vi "testUIPanelOpenifpreviouslyOpen.vi"(8 "error in (no error)":errorcluster, 11 "testStateMachineUtilities in":refnum<class "testStateMachineUtilities.lvclass">) -> (0 "error out":errorcluster, 3 "testStateMachineUtilities out":refnum<class "testStateMachineUtilities.lvclass">)   [LabVIEW 2020, in "testStateMachineUtilities.lvclass"]
uses:
  testStateMachineUtilities.lvclass
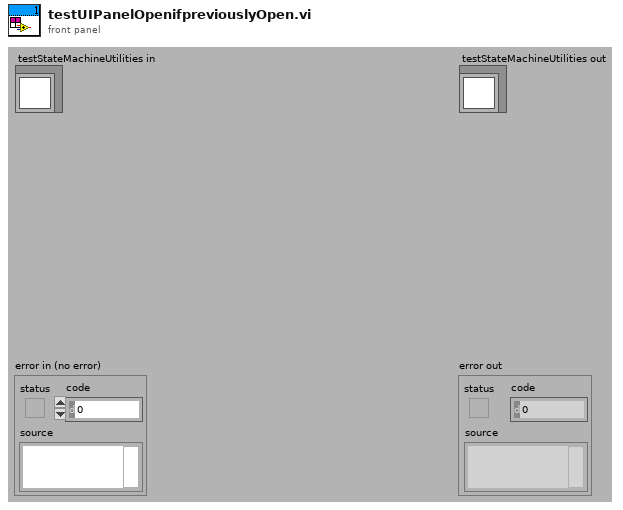
[diagram p1: front panel]
types:
  T1 = enum32{"Bad", "Idle", "Run top level", "Running"}
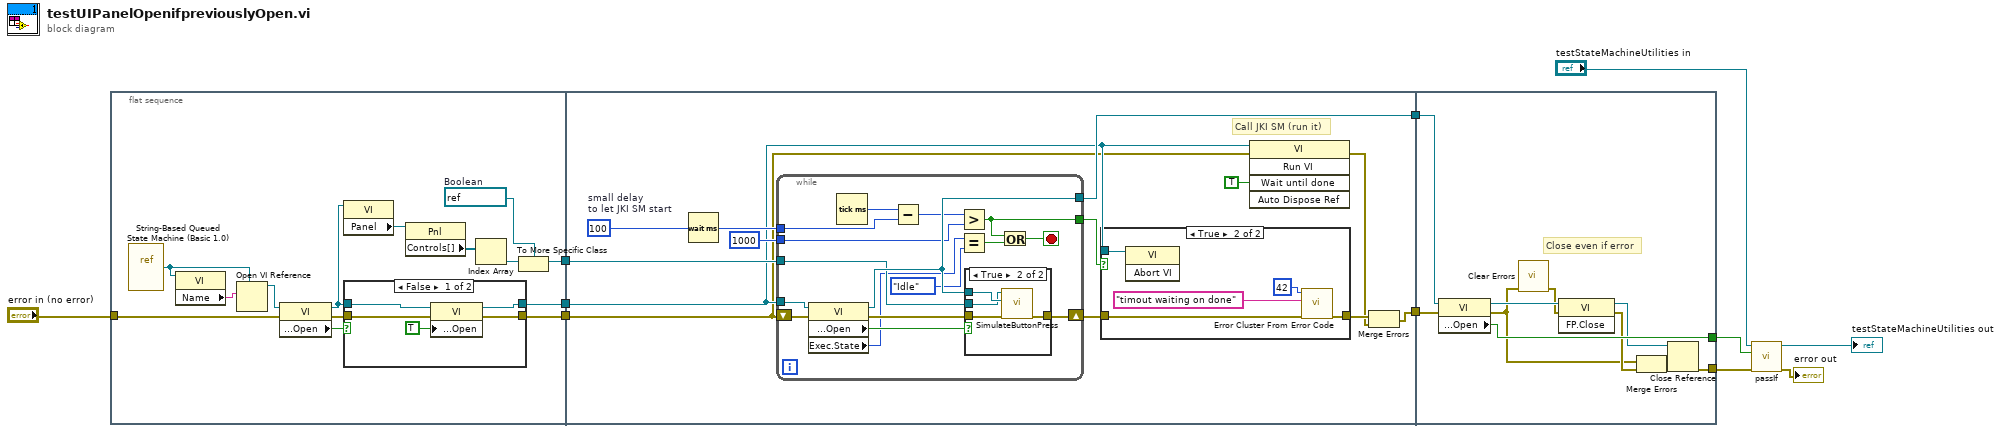
[diagram p0: block diagram]
diagram:
  n1 = flat-sequence {
    tunnel: [w23] -> w8
    tunnel: [w22] -> w3
    tunnel: "error in (no error)" -> [w21]
    tunnel: [w15] -> w1
    tunnel: w8 -> [w37]
    tunnel: [w45] -> w7
    tunnel: [w34] -> w4
    tunnel: w3 -> [w35]
    tunnel: w1 -> [w44]
    tunnel: w7 -> [w82]
    tunnel: [w80] -> w6
    tunnel: [w76] -> w5
    tunnel: w4 -> [w81]
    frame #0 {
      w16 = refnum<vi> refnum  # Boolean
      n2 = vi-ref "String-Based Queued State Machine (Basic 1.0).vi"() -> (w13:refnum<vi>)
      n3 = property class="VI"(reference=w13) -> ("Name"=w14:string)  [unwired: 1 in, 2 out]
      n4 = Open VI Reference(type specifier VI Refnum (for type only)=w13, vi path=w14) -> (vi reference=w12:refnum<vi>)  [unwired: 4 in, 1 out]
      n5 = property class="VI"(reference=w12, error in=w21) -> (reference out=w20:refnum<vi>, error out=w25:errorcluster, "Front Panel.Open"=w24:bool)
      n6 = property class="VI"(reference=w20) -> ("Panel"=w19:refnum<vi>)  [unwired: 1 in, 2 out]
      n7 = case shown="False" w24 {
        tunnel: w20 -> [w30 w32]
        tunnel: w25 -> [w28 w31]
        tunnel: [w27 w32] -> w23
        tunnel: [w26 w31] -> w22
        frame False {
          n8 = property class="VI"(reference=w30, error in=w28, "Front Panel.Open"=TRUE ("Front Panel Window:Open")) -> (reference out=w27:refnum<vi>, error out=w26:errorcluster)
        }
        frame True {
        }
      }
      n9 = property class="Pnl"(reference=w19) -> ("Controls[]"=w18:refnum<vi>[])  [unwired: 1 in, 2 out]
      n10 = Index Array(array=w18) -> (element=w17:refnum<vi>)  [unwired: 1 in]
      n11 = To More Specific Class(target class=w16, reference=w17) -> (specific class reference=w15:refnum<vi>)  [unwired: 1 in, 1 out]
    }
    frame #1 {
      w43 = u32 100  # small delay to let JKI SM start
      # "Call JKI SM (run it)"
      n12 = Wait (ms)(milliseconds to wait=w43) -> (millisecond timer value=w42:u32)
      n13 = while {
        tunnel: w37 -> [w67]
        tunnel: [w63] -> w45
        shift-right: [w66] -> w39
        shift-left: w35 -> [w65]
        tunnel: w44 -> [w62]
        tunnel: w42 -> [w60]
        tunnel: u32 1000 ("milliseconds to wait") -> [w58]
        tunnel: [w55] -> w40
        stop <- w56 stop-if-true
        n14 = property class="VI"(reference=w67, error in=w65) -> (reference out=w63:refnum<vi>, error out=w64:errorcluster, "Front Panel.Open"=w57:bool, "Exec.State"=w54:T1)
        n15 = Tick Count (ms)() -> (millisecond timer value=w61:u32)
        n16 = Subtract(x=w61, y=w60) -> (x-y=w59:u32)
        n17 = Greater?(x=w59, y=w58) -> (0:w55:bool)
        n18 = Equal?(x=w54, y=T1."Idle" ("Execution:State")) -> (x = y?=w52:bool)
        n19 = case shown="True" w57 {
          tunnel: [w68 w70] -> w66
          tunnel: w64 -> [w68 w69]
          tunnel: w63 -> [_ w72]
          tunnel: w62 -> [_ w71]
          frame False {
          }
          frame True {
            n20 = call "SimulateButtonPress.vi"("error in (no error)"=w69, "VIRef"=w72, "BooleanCtrlRef"=w71) -> ("error out"=w70:errorcluster)  [unwired: 8 in]
          }
        }
        n21 = Or(x=w55, y=w52) -> (x .or. y?=w56:bool)
      }
      n22 = case shown="True" w40 {
        tunnel: w37 -> [_ w51]
        tunnel: w39 -> [w46 w50]
        tunnel: [w46 w49] -> w38
        frame False {
        }
        frame True {
          n23 = invoke class="VI" method="Abort VI"(reference=w51) -> ()  [unwired: 2 in, 3 out]
          n24 = call <vilib>:"Error Cluster From Error Code.vi"("error in (no error)"=w50, "error message (\"\")"="timout waiting on done" ("error message (\"\")"), "error code (0)"=42) -> ("error out"=w49:errorcluster)  [unwired: 6 in]
        }
      }
      n25 = invoke class="VI" method="Run VI"(reference=w37, error in=w35, "Wait until done"=TRUE ("Wait Until Done")) -> (error out=w33:errorcluster)  [unwired: 2 in, 4 out]
      n26 = Merge Errors(w38, w33) -> (w34:errorcluster)
    }
    frame #2 {
      # "Close even if error"
      n27 = property class="VI"(reference=w82, error in=w81) -> (reference out=w79:refnum<vi>, error out=w74:errorcluster, "Front Panel.Open"=w80:bool)
      n28 = call <vilib>:"Clear Errors.vi"("error in (no error)"=w74) -> ("error out"=w73:errorcluster)  [unwired: 5 in, 1 out]
      n29 = invoke class="VI" method="FP.Close"(reference=w79, error in=w73) -> (reference out=w78:refnum<vi>, error out=w77:errorcluster)  [unwired: 1 in, 1 out]
      n30 = Merge Errors(w74, w77) -> (w75:errorcluster)
      n31 = Close Reference(reference=w78, error in (no error)=w75) -> (error out=w76:errorcluster)
    }
  }
  n32 = call-dynamic "passIf.vi"("error in (no error)"=w5, "pass"=w6, "TestCase in"="testStateMachineUtilities in") -> ("error out"=→"error out":errorcluster, "TestCase out"=→"testStateMachineUtilities out":refnum<class "testStateMachineUtilities.lvclass">)  [unwired: 7 in]
